vi "Update Message Getter.vi"(7 "rpc message name":string, 8 "error in (no error)":errorcluster, 10 "message getter in":refnum<vi>, 11 "rpc messages folder in":refnum<vi>) -> (0 "error out":errorcluster, 2 "message getter out":refnum<vi>, 3 "rpc messages folder out":refnum<vi>)   [LabVIEW 2019, in "gRPC Template Creation Utility.lvlib"]
uses:
  gRPC Template Creation Utility.lvlib
  Oneof API/OneOf Constants/OneOfConstantsEnum.ctl
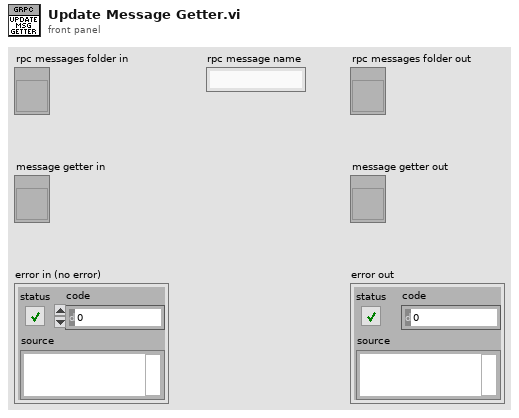
[diagram p1: front panel]
types:
  T1 = typedef "gRPC Template Creation Utility.lvlib/OneOfConstantsEnum.ctl" = enum16{"FlatToRichVIPrefix", "RichToFlatVIPrefix", "FlatTypeDefSuffix"}
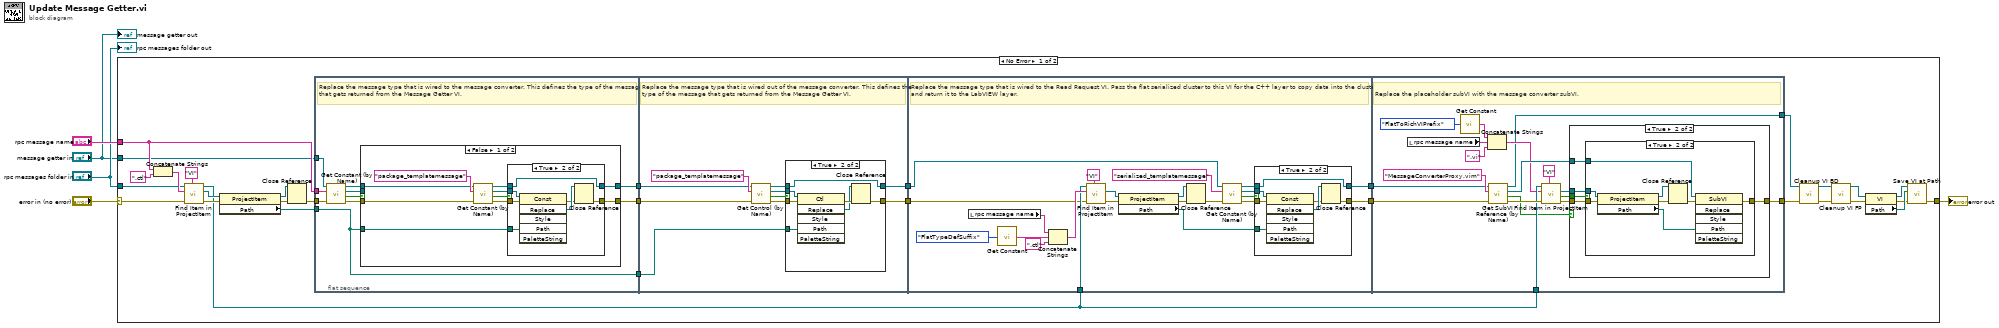
[diagram p0: block diagram]
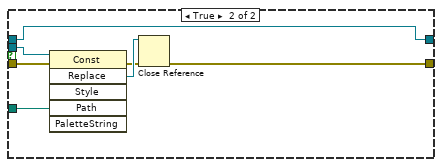
[diagram p3: hidden frame]
diagram:
  n1 = case shown="No Error" "error in (no error)" {
    selector: "error in (no error)" -> [w23 w156]
    tunnel: [w21 w156] -> w5
    tunnel: "rpc message name" -> [w24 _]
    tunnel: "rpc messages folder in" -> [w22 _]
    tunnel: "message getter in" -> [w19 _]
    frame No Error {
      n2 = Concatenate Strings(w24, ".ctl" ("string")) -> (w30:string)
      n3 = call "Find Item in ProjectItem.vi"("Item Type"="VI", "error in (no error)"=w23, "Name"=w30, "ProjectItem in"=w22) -> ("error out"=w34:errorcluster, "Item Refnum out"=w33:refnum<vi>, "ProjectItem out"=w13:refnum<vi>)  [unwired: 4 in, 1 out]
      n4 = property class="ProjectItem"(reference=w33, error in=w34) -> (reference out=w35:refnum<vi>, error out=w36:errorcluster, "Path"=w28:path)
      n5 = Close Reference(reference=w35, error in (no error)=w36) -> (error out=w20:errorcluster)
      n6 = flat-sequence {
        tunnel: w28 -> [w37]
        tunnel: w20 -> [w45]
        tunnel: w24 -> [w44]
        tunnel: [w46] -> w29
        tunnel: w19 -> [w39]
        tunnel: [w38] -> w15
        tunnel: [w37] -> w12
        tunnel: w29 -> [w78]
        tunnel: [w77] -> w27
        tunnel: [w73] -> w26
        tunnel: w15 -> [w76]
        tunnel: w12 -> [w75]
        tunnel: w27 -> [w99]
        tunnel: w26 -> [w96]
        tunnel: [w113] -> w25
        tunnel: w13 -> [w101]
        tunnel: [w92] -> w14
        tunnel: w25 -> [w127]
        tunnel: w13 -> [w136]
        tunnel: [w133] -> w11
        tunnel: w14 -> [w134]
        tunnel: [w125] -> w8
        frame #0 {
          # "Replace the message type that is wired to the message converter. This defines the type of the message that gets returned from the Message Getter VI."
          n7 = call "Get Constant (by Name).vi"("error in (no error)"=w45, "Constant Label"=w44, "Owner VI in"=w39) -> ("error out"=w43:errorcluster, "Found ?"=w42:bool, "Const ref out"=w41:refnum<vi>, "Owner VI out"=w40:refnum<vi>)  [unwired: 5 in]
          n8 = case shown="False" w42 {
            tunnel: [w56 w67] -> w46
            tunnel: w37 -> [w55 w68]
            tunnel: w43 -> [w50 w72]
            tunnel: w40 -> [w49 w66]
            tunnel: w41 -> [_ w71]
            tunnel: [w47 w66] -> w38
            frame False {
              n9 = call "Get Constant (by Name).vi"("error in (no error)"=w50, "Constant Label"="package_templatemessage" ("name/order"), "Owner VI in"=w49) -> ("error out"=w52:errorcluster, "Found ?"=w51:bool, "Const ref out"=w54:refnum<vi>, "Owner VI out"=w48:refnum<vi>)  [unwired: 5 in]
              n10 = case shown="True" w51 {
                tunnel: [w58 w65] -> w56
                tunnel: w55 -> [_ w64]
                tunnel: w54 -> [_ w61]
                tunnel: w52 -> [w58 w60]
                tunnel: w48 -> [w57 w59]
                tunnel: [w57 w59] -> w47
                frame False {
                }
                frame True {
                  n11 = invoke class="Const" method="Replace"(reference=w61, error in=w60, "Path"=w64) -> (error out=w62:errorcluster, "Replace"=w63:refnum<vi>)  [unwired: 3 in, 4 out]
                  n12 = Close Reference(reference=w63, error in (no error)=w62) -> (error out=w65:errorcluster)
                }
              }
            }
            frame True {
              n13 = invoke class="Const" method="Replace"(reference=w71, error in=w72, "Path"=w68) -> (error out=w69:errorcluster, "Replace"=w70:refnum<vi>)  [unwired: 3 in, 4 out]
              n14 = Close Reference(reference=w70, error in (no error)=w69) -> (error out=w67:errorcluster)
            }
          }
        }
        frame #1 {
          # "Replace the message type that is wired out of the message converter. This defines the type of the message that gets returned from the Message Getter VI."
          n15 = call "Get Control (by Name).vi"("error in (no error)"=w78, "Control Label"="package_templatemessage" ("name/order"), "Owner VI in"=w76) -> ("error out"=w82:errorcluster, "Found ?"=w81:bool, "Control Refnum"=w80:refnum<vi>, "Owner VI out"=w74:refnum<vi>)  [unwired: 5 in]
          n16 = case shown="True" w81 {
            tunnel: [w84 w91] -> w77
            tunnel: w75 -> [_ w88]
            tunnel: w80 -> [_ w87]
            tunnel: w82 -> [w84 w86]
            tunnel: w74 -> [w83 w85]
            tunnel: [w83 w85] -> w73
            frame False {
            }
            frame True {
              n17 = invoke class="Ctl" method="Replace"(reference=w87, error in=w86, "Path"=w88) -> (error out=w90:errorcluster, "Replace"=w89:refnum<vi>)  [unwired: 3 in, 4 out]
              n18 = Close Reference(reference=w89, error in (no error)=w90) -> (error out=w91:errorcluster)
            }
          }
        }
        frame #2 {
          # "Replace the message type that is wired to the Read Request VI. Pass the flat serialized cluster to this VI for the C++ layer to copy data into the cluster and return it to the LabVIEW layer."
          n19 = local read "rpc message name"() -> (w97:string)
          n20 = call "Get Constant.vi"("Selection"=OneOfConstantsEnum."FlatTypeDefSuffix") -> ("String"=w94:string)
          n21 = Concatenate Strings(w97, w94, ".ctl" ("string")) -> (w104:string)
          n22 = call "Find Item in ProjectItem.vi"("Item Type"="VI", "error in (no error)"=w99, "Name"=w104, "ProjectItem in"=w101) -> ("error out"=w106:errorcluster, "Item Refnum out"=w105:refnum<vi>)  [unwired: 4 in, 2 out]
          n23 = property class="ProjectItem"(reference=w105, error in=w106) -> (reference out=w107:refnum<vi>, error out=w108:errorcluster, "Path"=w100:path)
          n24 = Close Reference(reference=w107, error in (no error)=w108) -> (error out=w98:errorcluster)
          n25 = call "Get Constant (by Name).vi"("error in (no error)"=w98, "Constant Label"="serialized_templatemessage" ("name/order"), "Owner VI in"=w96) -> ("error out"=w112:errorcluster, "Found ?"=w111:bool, "Const ref out"=w110:refnum<vi>, "Owner VI out"=w93:refnum<vi>)  [unwired: 5 in]
          n26 = case shown="True" w111 {
            tunnel: [w115 w117] -> w113
            tunnel: w100 -> [_ w118]
            tunnel: w112 -> [w115 w122]
            tunnel: w110 -> [_ w121]
            tunnel: w93 -> [w114 w116]
            tunnel: [w114 w116] -> w92
            frame False {
            }
            frame True {
              n27 = invoke class="Const" method="Replace"(reference=w121, error in=w122, "Path"=w118) -> (error out=w119:errorcluster, "Replace"=w120:refnum<vi>)  [unwired: 3 in, 4 out]
              n28 = Close Reference(reference=w120, error in (no error)=w119) -> (error out=w117:errorcluster)
            }
          }
        }
        frame #3 {
          # "Replace the placeholder subVI with the message converter subVI."
          n29 = local read "rpc message name"() -> (w126:string)
          n30 = call "Get Constant.vi"("Selection"=OneOfConstantsEnum."FlatToRichVIPrefix") -> ("String"=w123:string)
          n31 = Concatenate Strings(w123, w126, ".vi" ("string")) -> (w128:string)
          n32 = call "Get SubVI Reference (by Name).vi"("error in (no error)"=w127, "SubVI Name"="MessageConverterProxy.vim", "Owner VI in"=w134) -> ("error out"=w139:errorcluster, "Found ?"=w131:bool, "SubVI Refnum out"=w132:refnum<vi>, "Owner VI out"=w125:refnum<vi>)  [unwired: 5 in]
          n33 = call "Find Item in ProjectItem.vi"("Item Type"="VI", "error in (no error)"=w139, "Name"=w128, "ProjectItem in"=w136) -> ("error out"=w140:errorcluster, "Found ?"=w130:bool, "Item Refnum out"=w138:refnum<vi>)  [unwired: 4 in, 1 out]
          n34 = case shown="True" w131 {
            tunnel: w138 -> [_ w146]
            tunnel: [w141 w145] -> w133
            tunnel: w140 -> [w141 w144]
            tunnel: w132 -> [_ w143]
            tunnel: w130 -> [_ w142]
            frame False {
            }
            frame True {
              n35 = case shown="True" w142 {
                tunnel: w146 -> [_ w155]
                tunnel: [w147 w148] -> w145
                tunnel: w144 -> [w147 w153]
                tunnel: w143 -> [_ w151]
                frame False {
                }
                frame True {
                  n36 = property class="ProjectItem"(reference=w155, error in=w153) -> (reference out=w152:refnum<vi>, error out=w150:errorcluster, "Path"=w154:path)
                  n37 = Close Reference(reference=w152, error in (no error)=w150) -> (error out=w149:errorcluster)
                  n38 = invoke class="SubVI" method="Replace"(reference=w151, error in=w149, "Path"=w154) -> (error out=w148:errorcluster)  [unwired: 3 in, 5 out]
                }
              }
            }
          }
        }
      }
      n39 = call "Cleanup VI BD.vi"("error in (no error)"=w11, "VI in"=w8) -> ("error out"=w10:errorcluster, "VI out"=w7:refnum<vi>)  [unwired: 8 in]
      n40 = call "Cleanup VI FP.vi"("error in"=w10, "vi in"=w7) -> ("error out"=w9:errorcluster, "vi out"=w6:refnum<vi>)  [unwired: 8 in]
      n41 = property class="VI"(reference=w6, error in=w9) -> (reference out=w17:refnum<vi>, error out=w16:errorcluster, "Path"=w18:path)
      n42 = call "Save VI at Path.vi"("error in (no error)"=w16, "Path"=w18, "VI in"=w17) -> ("error out"=w21:errorcluster)  [unwired: 6 in, 2 out]
    }
    frame Error {
    }
  }
  "error out" <- w5
  "rpc messages folder out" <- "rpc messages folder in"
  "message getter out" <- "message getter in"
